vi "ProcCore.vi"(7 "ProcessParams":T1={"DisplayIncrement"=0, "DisplayIncrementRef"=refnum, "Rep .Rate (Hz)"=10.0, "Save"=FALSE, "SW_Average"=0, "Filter"=enum."None", "FilterParams"=variant, "DAQParams"={"TrigDelay"=0.0, "Offset"=0, "Resolution"=-32768, "Range (mV)"=0, "Sample Rate"=100000000.0, "Depth"=16384.0, "Segments"=1}, "Graph"=[], "CmdParams."=variant, "Average(SW)Ref"=refnum, "Calibr.Params"=refnum, "SignalSegmentRef"=refnum, "WriterQueue"=refnum} {"DAQParams"."Segments" min=1 max=1024 step=1; "DAQParams"."Sample Rate" format="%.0p"}, 8 "error in":errorcluster, 9 "SignalBuffer in":refnum<queue>, 10 "CtrlQueue in":refnum<queue>) -> (0 "error out":errorcluster)   [LabVIEW 2013]
uses:
  <instrlib>/AnalogDiscSDKLv/VIs/DWF_Signal.ctl
  ProcessParams.ctl
  ControlDef/ProcessingMode.ctl
  DAQParams.ctl
  DisplayGraph.ctl
  Binning/BinType.ctl
  ControlDef/Average#.ctl
  Files/Signal_Segment.ctl
  ControlDef/Signal.ctl
  ProcessStates.ctl
  <vilib>/Utility/error.llb/DialogType.ctl
  Binning/SpectrumBinning.vi
  MassResolutionCalc/FindMassResolution_Single.vi
  <instrlib>/AnalogDiscSDKLv/AnalogDiscSDKLv.lvlib
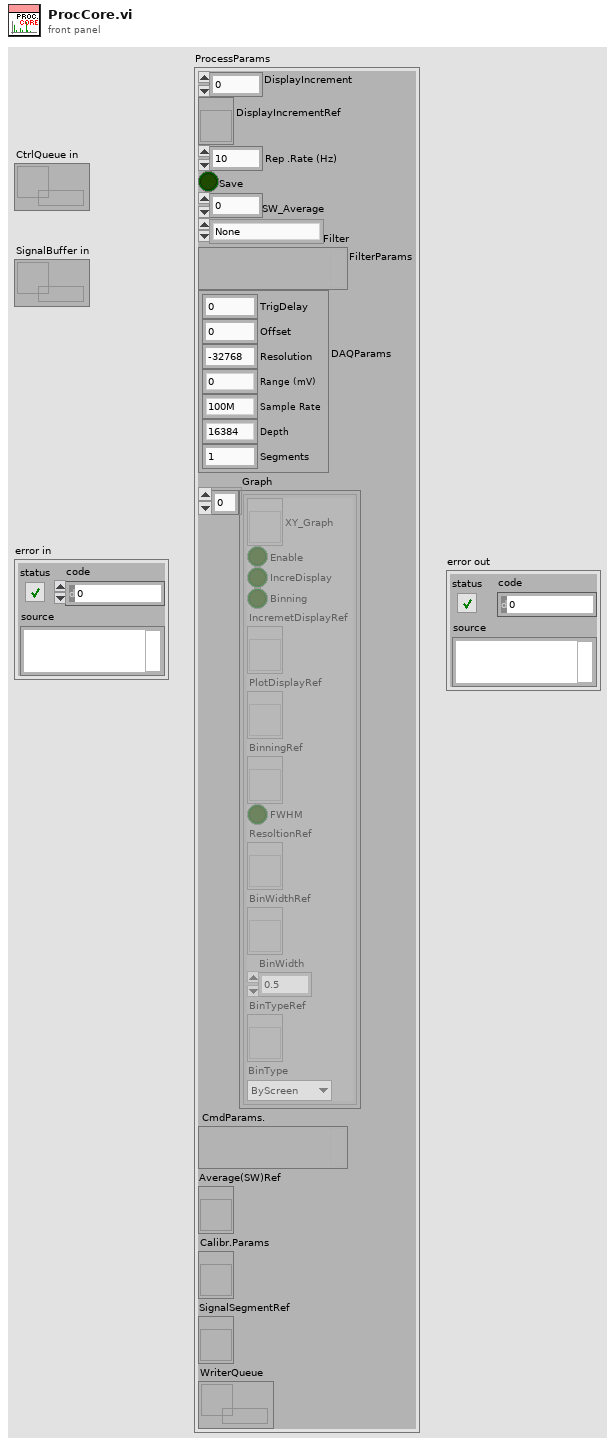
[diagram p1: front panel]
types:
  T1 = typedef "ProcessParams.ctl" = cluster{"DisplayIncrement":u32, "DisplayIncrementRef":refnum<vi>, "Rep .Rate (Hz)":dbl, "Save":bool, "SW_Average":u32, "Filter":T2, "FilterParams":variant, "DAQParams":T3, "Graph":T4[], "CmdParams.":variant, "Average(SW)Ref":refnum<vi>, "Calibr.Params":refnum<vi>, "SignalSegmentRef":refnum<vi>, "WriterQueue":refnum<queue>}
  T2 = typedef "ProcessingMode.ctl" = enum16{"None", "Drop by Threshold", "TDC Simulate", "SetFilter"}
  T3 = typedef "DAQParams.ctl" = cluster{"TrigDelay":dbl, "Offset":i32, "Resolution":i32, "Range (mV)":u32, "Sample Rate":dbl, "Depth":dbl, "Segments":u32}
  T4 = typedef "DisplayGraph.ctl" = cluster{"XY_Graph":refnum<vi>, "Enable":bool, "IncreDisplay":bool, "Binning":bool, "IncremetDisplayRef":refnum<vi>, "PlotDisplayRef":refnum<vi>, "BinningRef":refnum<vi>, "FWHM":bool, "ResoltionRef":refnum<vi>, "BinWidthRef":refnum<vi>, "BinWidth":dbl, "BinTypeRef":refnum<vi>, "BinType":T5}
  T5 = typedef "BinType.ctl" = enum16{"ByTime", "ByScreen", "ByMass", "ToUnitMass"}
  T6 = typedef "ProcessStates.ctl" = enum16{"Initialize", "Normal", "Display", "Write2Buffer", "CalcMzArray", "StartSave", "StopSave", "ConfigChanged", "EndOfLine", "SetFilterParams", "SetGraphsEnable", "SetAcquisitionParams", "ChangeDisplayIncrement", "ChangeRepRate", "SetWriterRef", "Quit", "StartOfLine"}
  T7 = typedef "Signal_Segment.ctl" = cluster{"SampleRate":dbl, "TrigDelay":dbl, "SpecLength":dbl, "DAQ_Range":dbl, "Average#":i32, "Position":dbl[], "Spectrum":sgl[], "Calibr.":dbl[], "Pressure":dbl, "Desp_LaserEnergy":dbl, "PI_LaserEnergy":dbl, "Voltages Table":sgl[][], "ProcMode":T2, "Threshold":dbl, "Comment":string, "TickCount":dbl, "Time Stamp":timestamp}
  T8 = typedef "Average#.ctl" = u16
  T9 = typedef "Signal.ctl" = cluster{"Command":T6, "Params":variant}
  T10 = typedef "AnalogDiscSDKLv.lvlib/DWF_Signal.ctl" = cluster{"tickcount":u32, "Signal":sgl[][], "SecondaryData":dbl[], "Flag":enum16{"Normal", "MultiRecStart", "MultiRecEnd", "Reserved1", "Reserved2", "Reserved3"}}
  T11 = enum16{"Normal", "MultiRecStart", "MultiRecEnd", "Reserved1", "Reserved2", "Reserved3"}
  T12 = typedef "DialogType.ctl" = u16
  T13 = cluster{"WriterQueue":refnum<queue>, "feedback queue":refnum<queue>}
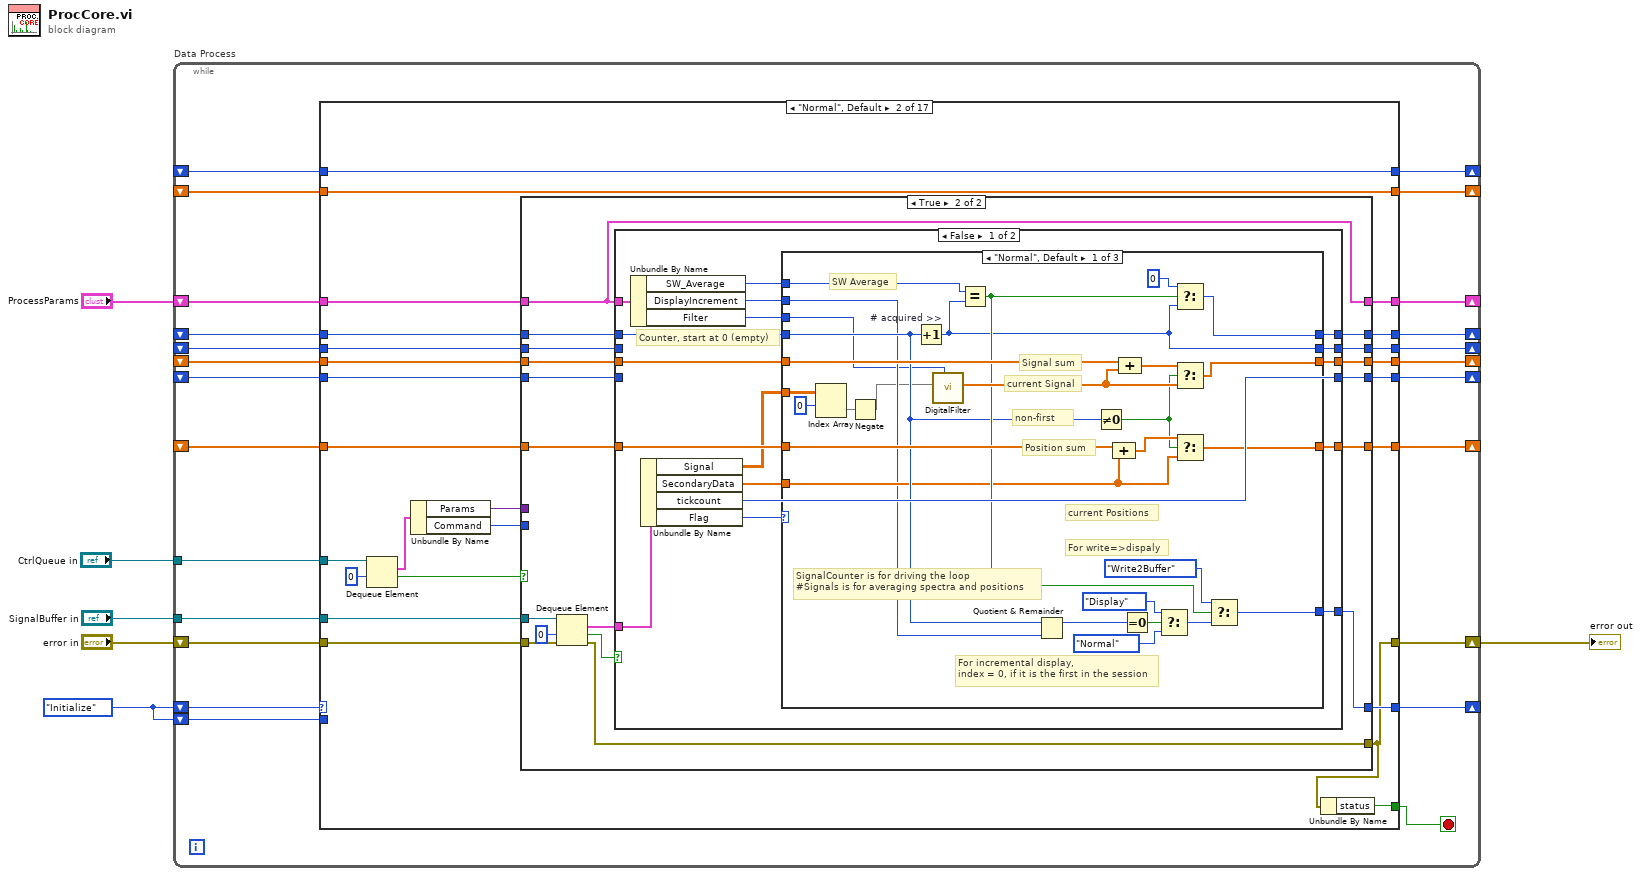
[diagram p0: block diagram]
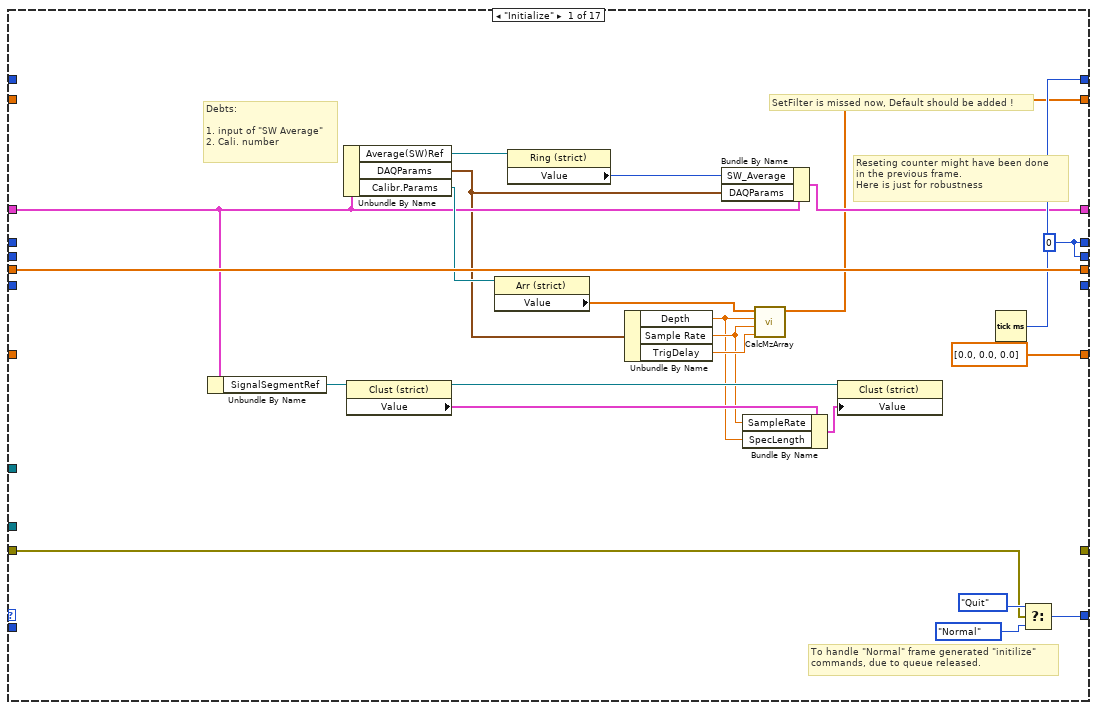
[diagram p2: hidden frame]
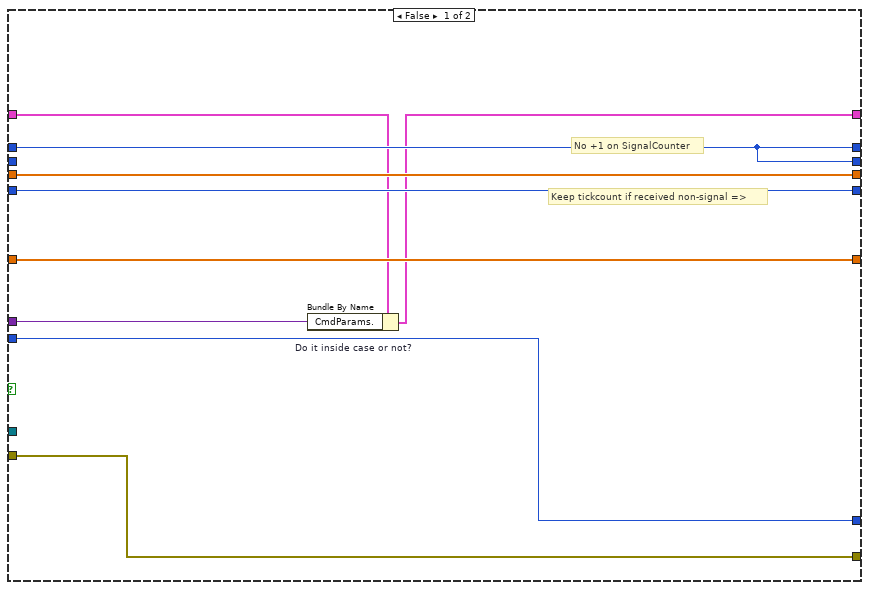
[diagram p3: hidden frame]
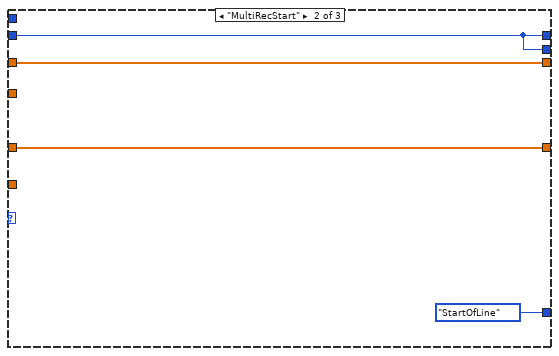
[diagram p4: hidden frame]
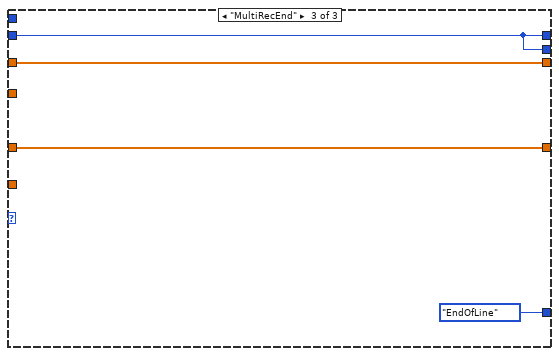
[diagram p5: hidden frame]
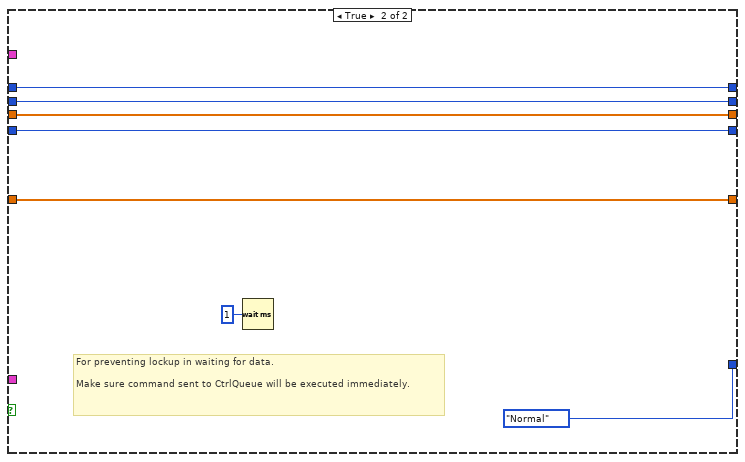
[diagram p6: hidden frame]
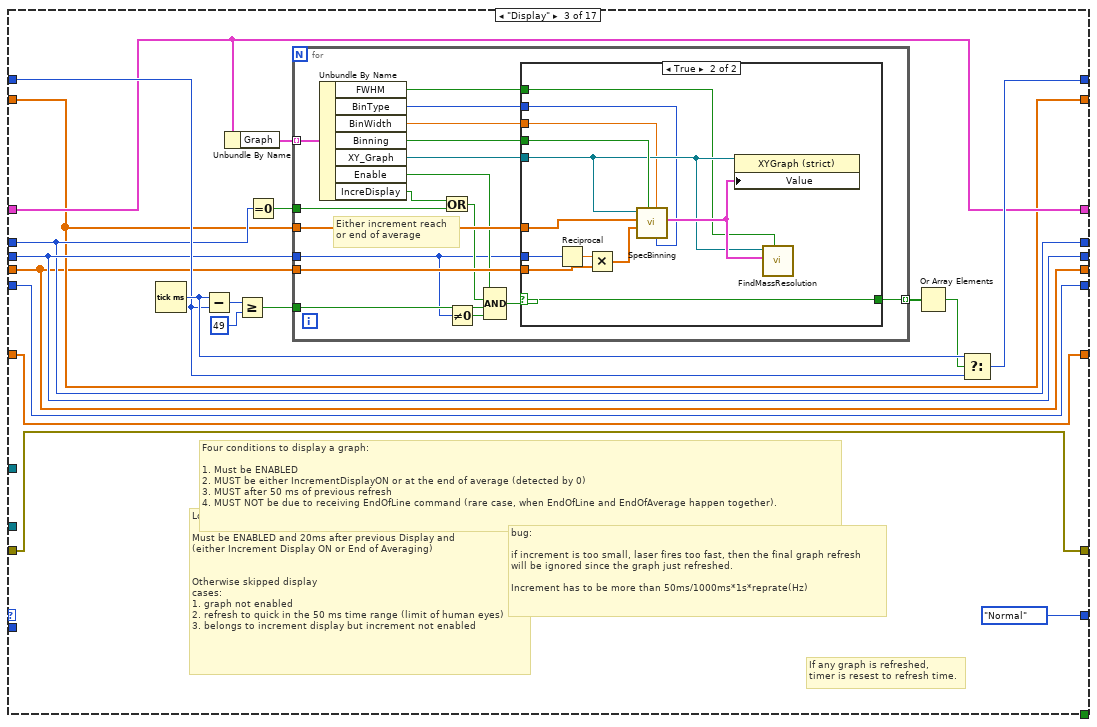
[diagram p7: hidden frame]
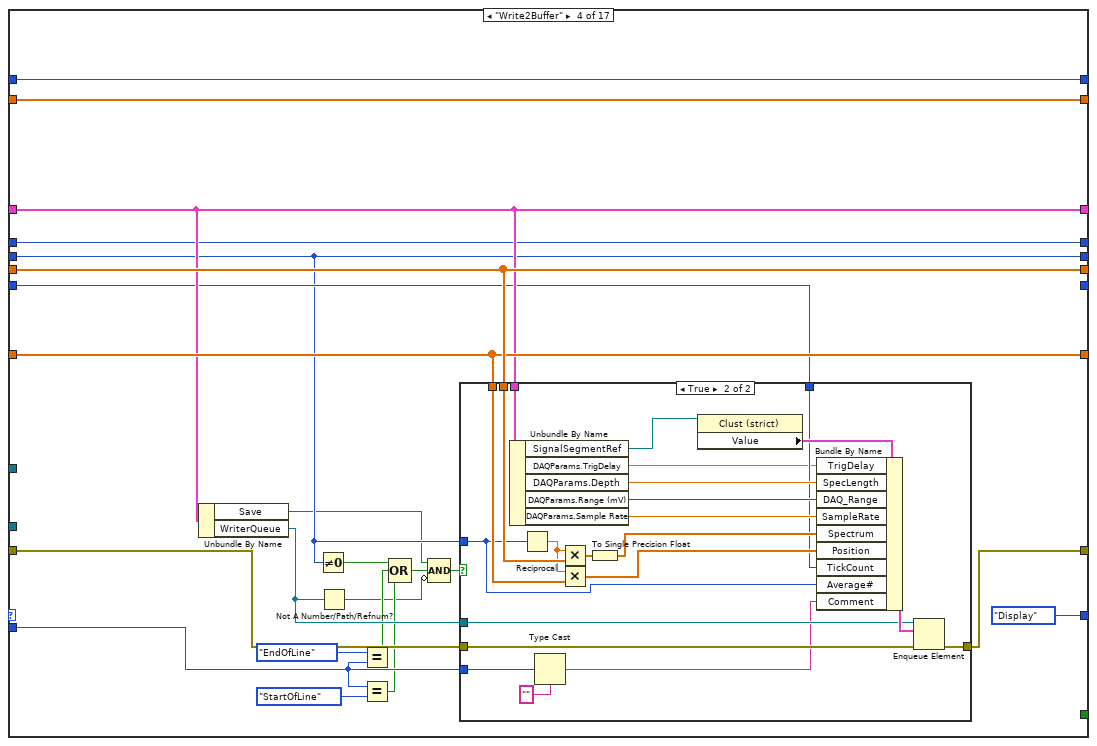
[diagram p9: hidden frame]
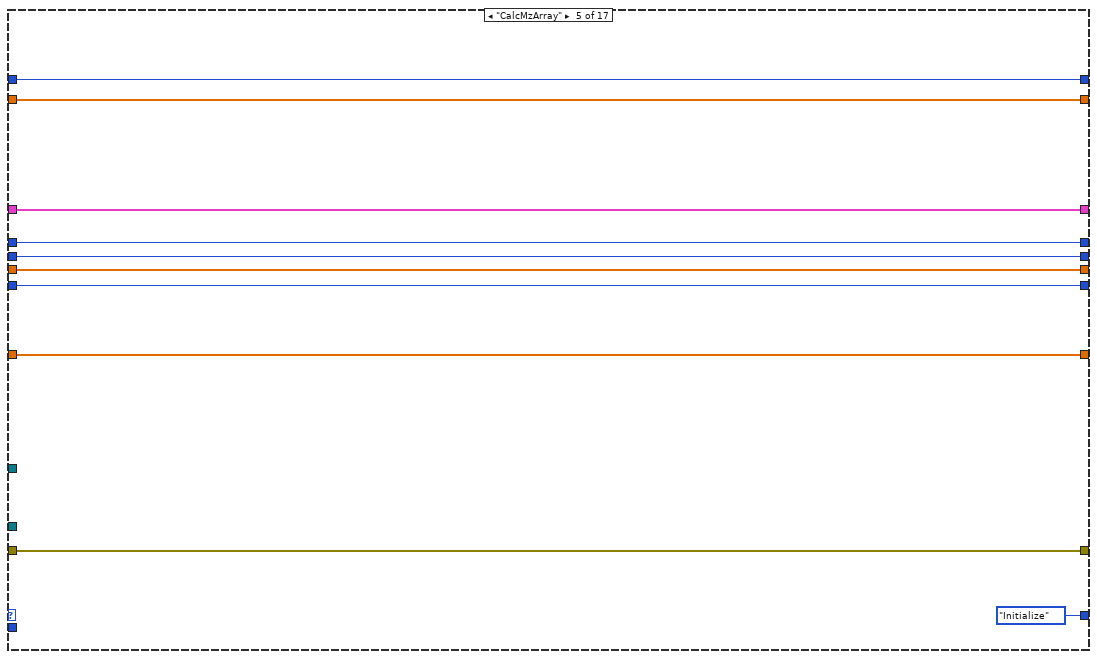
[diagram p11: hidden frame]
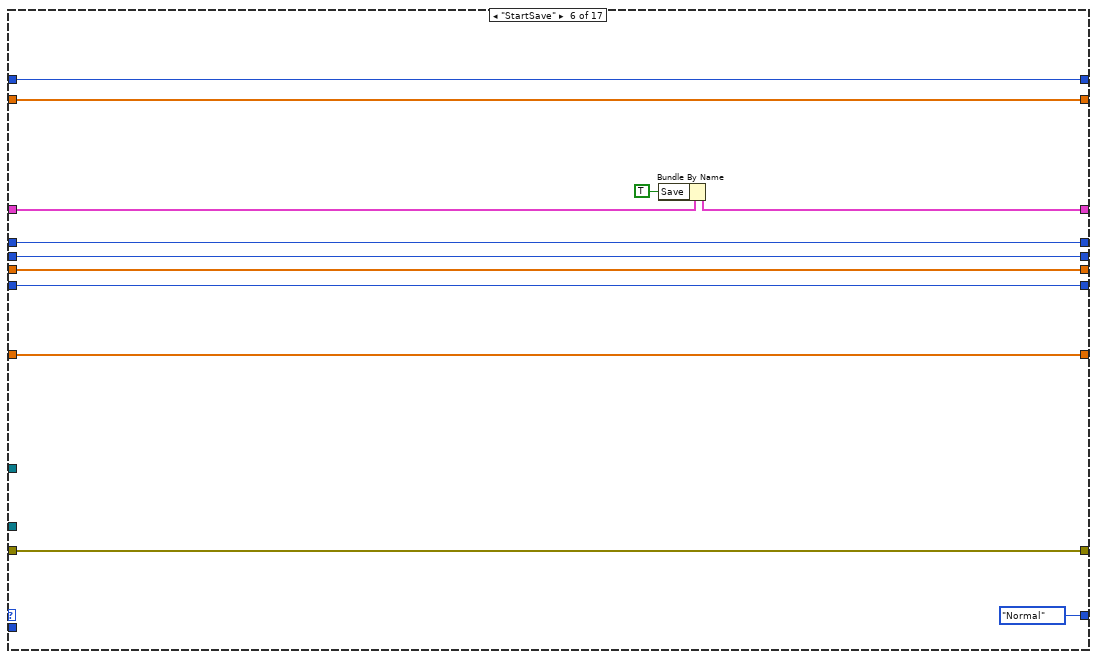
[diagram p12: hidden frame]
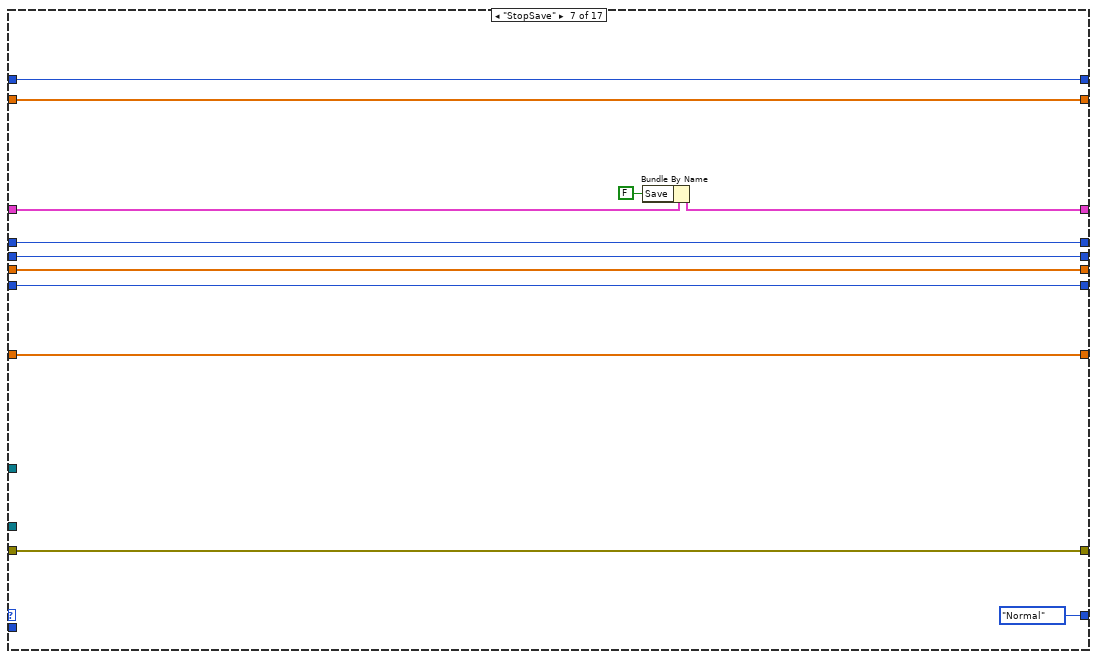
[diagram p13: hidden frame]
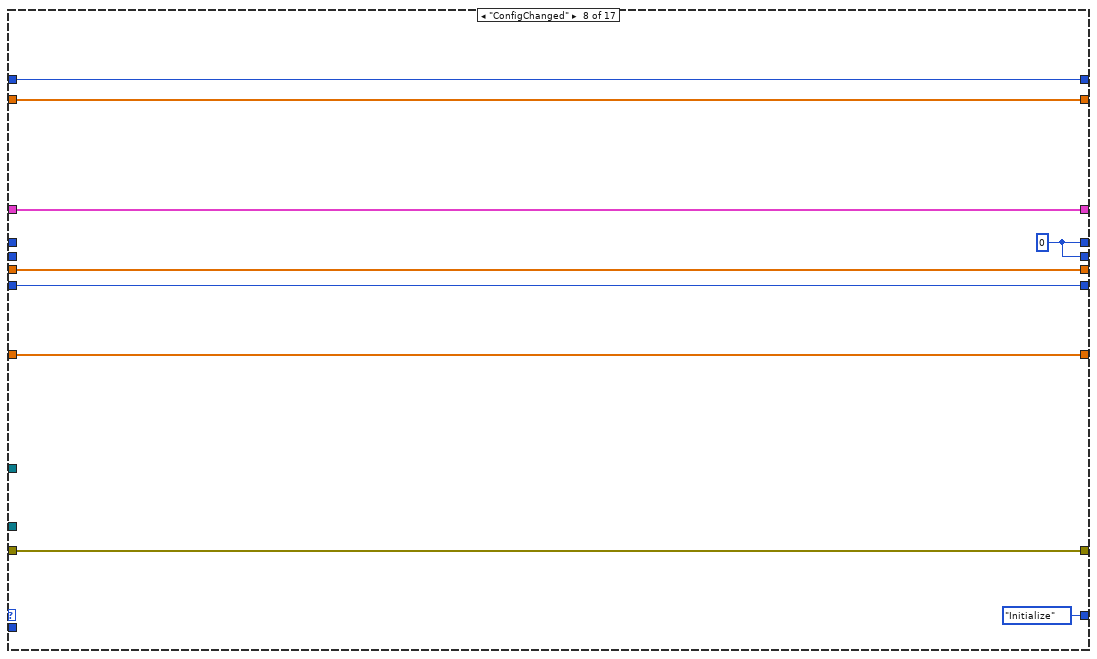
[diagram p14: hidden frame]
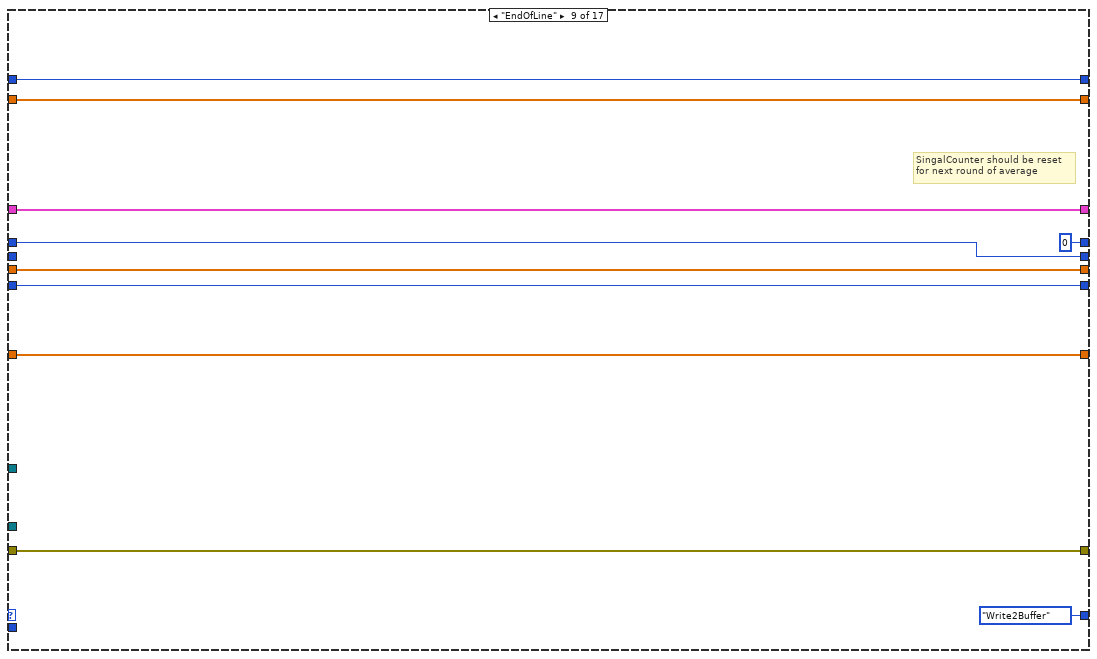
[diagram p15: hidden frame]
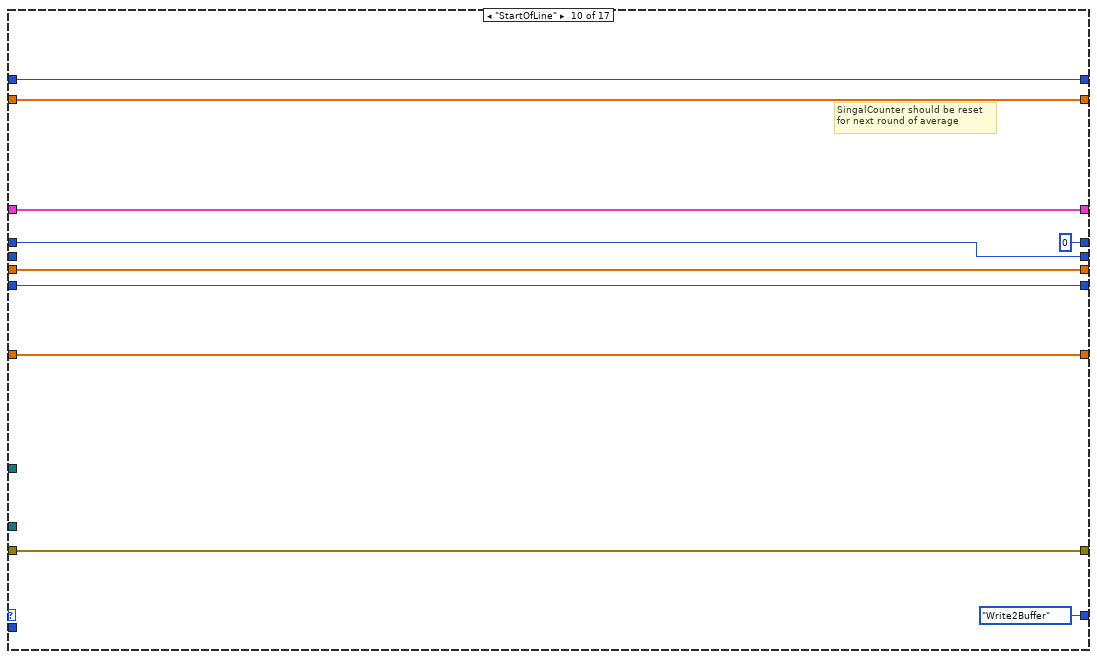
[diagram p16: hidden frame]
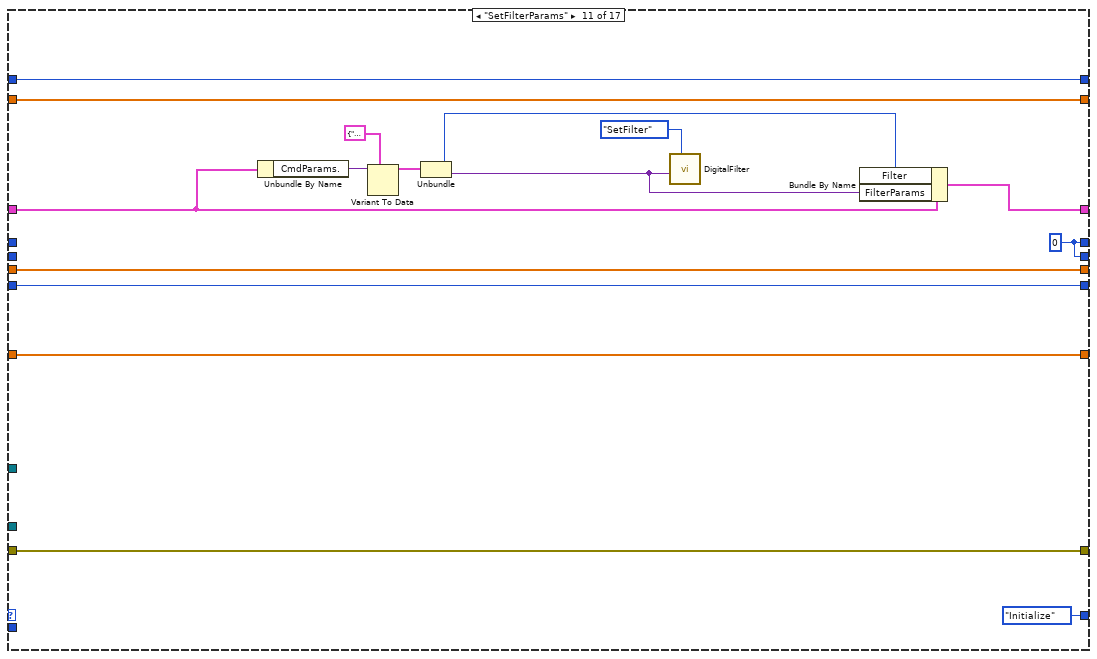
[diagram p17: hidden frame]
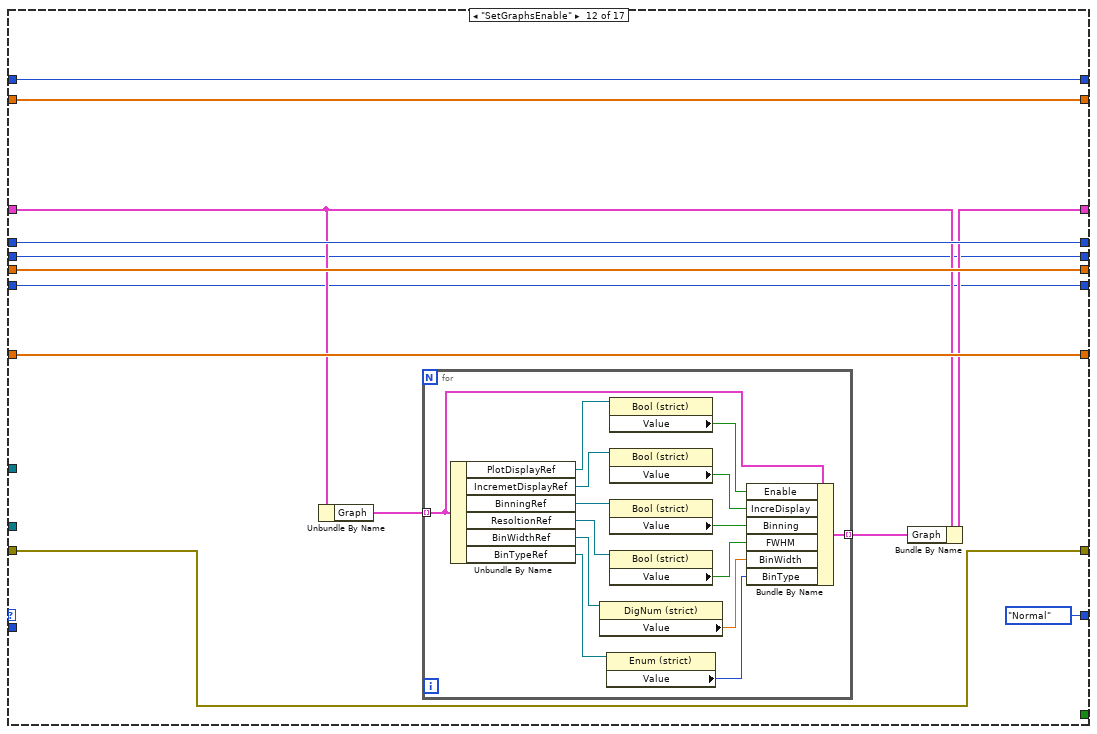
[diagram p18: hidden frame]
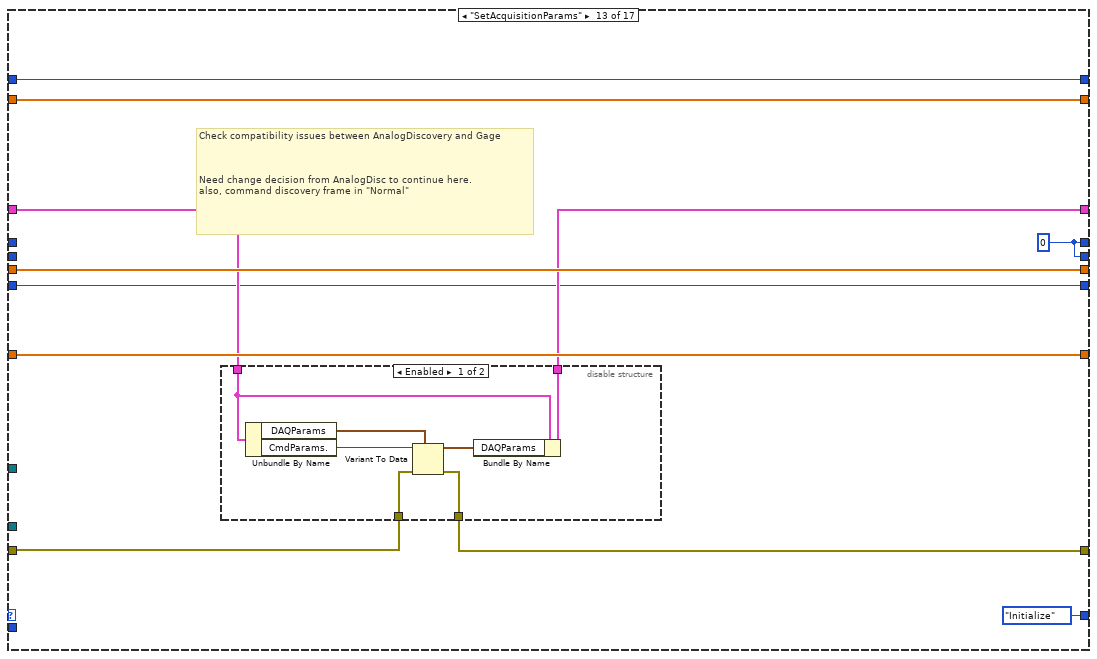
[diagram p19: hidden frame]
diagram:
  w3 = ProcessStates."Initialize"
  n1 = while "Data Process" {
    tunnel: "SignalBuffer in" -> [w30]
    shift-right: [w24] -> _
    shift-left: _ -> [w28]
    shift-right: [w26] -> _
    shift-left: _ -> [w27]
    shift-right: [w25] -> w4
    shift-left: "error in" -> [w29]
    shift-right: [w16] -> _
    shift-left: _ -> [w22]
    shift-right: [w17] -> _
    shift-left: _ -> [w21]
    shift-right: [w14] -> _
    shift-left: _ -> [w15]
    shift-right: [w19] -> _
    shift-left: "ProcessParams" -> [w20]
    shift-right: [w18] -> _
    shift-left: w3 -> [w13]
    shift-left: w3 -> [w12]
    shift-right: [w11] -> _
    shift-left: _ -> [w10]
    shift-right: [w9] -> _
    shift-left: _ -> [w8]
    tunnel: "CtrlQueue in" -> [w7]
    stop <- w23 stop-if-true
    n2 = case shown="\"Normal\", Default" w13 {
      tunnel: w30 -> [_ w60 _ _ _ _ _ _ _ _ _ _ _ _ _ _ _]
      tunnel: w29 -> [w41 w58 w184 w233 w267 w279 w291 w300 w310 w320 w336 w349 w369 w401 w427 w452 w474]
      tunnel: w28 -> [w53 w74 w166 w231 w266 w278 w290 w299 w309 w319 w335 w348 w374 w400 w426 w457 w481]
      tunnel: w27 -> [_ w78 w180 w230 w268 w280 w292 w301 w311 w321 w337 w350 w375 w402 w428 w458 w482]
      tunnel: [dbl[] [0.0, 0.0, 0.0] w72 w180 w230 w268 w280 w292 w301 w311 w321 w337 w350 w375 w402 w428 w458 w482] -> w26
      tunnel: [_ w59 w184 w232 w267 w279 w291 w300 w310 w320 w336 w349 w368 w401 w427 w442 w474] -> w25
      tunnel: [w53 w75 w166 w231 w266 w278 w290 w299 w309 w319 w335 w348 w374 w400 w426 w457 w481] -> w24
      tunnel: [_ w69 _ _ _ _ _ _ _ _ _ _ _ _ _ _ TRUE] -> w23
      tunnel: w22 -> [_ w77 w176 w235 w264 w275 w287 w297 w307 w317 w334 w346 w373 w398 w424 w456 w478]
      tunnel: w21 -> [_ w70 w170 w227 w265 w276 w288 _ w304 w314 _ w347 _ w399 w425 _ w479]
      tunnel: w15 -> [_ w76 w167 w234 w261 w274 w286 w296 w306 w316 w333 w345 w372 w397 w423 w455 w477]
      tunnel: w20 -> [w40 w56 w169 w228 w262 w277 w289 w298 w308 w318 w329 w342 w367 w394 w420 w451 w480]
      tunnel: [w49 w55 w169 w228 w262 w273 w285 w298 w308 w318 w332 w344 w370 w393 w415 w453 w480] -> w19
      tunnel: [w42 w73 ProcessStates."Normal" ProcessStates."Display" ProcessStates."Initialize" ProcessStates."Normal" ProcessStates."Normal" ProcessStates."Initialize" ProcessStates."Write2Buffer" ProcessStates."Write2Buffer" ProcessStates."Initialize" ProcessStates."Normal" ProcessStates."Initialize" ProcessStates."Normal" ProcessStates."Normal" ProcessStates."Normal" ProcessStates."Quit"] -> w18
      tunnel: [w33 w71 w170 w227 w265 w276 w288 w294 u32 0 ("t") u32 0 ("t") w323 w347 w366 w399 w425 w450 w479] -> w17
      tunnel: [w51 w77 w177 w235 w264 w275 w287 w297 w307 w317 w334 w346 w373 w398 w424 w456 w478] -> w16
      tunnel: [w32 w76 w167 w234 w261 w274 w286 w296 w306 w316 w333 w345 w372 w397 w423 w455 w477] -> w14
      tunnel: w12 -> [_ _ _ w219 _ _ _ _ _ _ _ _ _ _ _ _ _]
      tunnel: [w33 w68 w172 w225 w260 w270 w282 w294 w304 w314 w323 w339 w366 w396 w422 w450 w473] -> w11
      tunnel: w10 -> [_ w54 w172 w225 w260 w270 w282 _ _ _ _ w339 _ w396 w422 _ w473]
      tunnel: [_ w67 w168 _ w259 w269 w281 w293 w302 w312 w322 w338 w365 w392 w418 w449 _] -> w9
      tunnel: w8 -> [_ w66 w168 w226 w259 w269 w281 w293 w302 w312 w322 w338 w365 w392 w418 w449 _]
      tunnel: w7 -> [_ w64 _ _ _ _ _ _ _ _ _ _ _ _ _ _ _]
      frame "Initialize" {
        w33 = u32 0 ("t")
        # "SetFilter is missed now, Default should be added !"
        # "Reseting counter might have been done\nin the previous frame.\nHere is just for robustness"
        # "To handle \"Normal\" frame generated \"initilize\"\ncommands, due to queue released."
        # "Debts:\n\n1. input of \"SW Average\"\n2. Cali. number"
        n3 = Unbundle By Name(w40) -> ("SignalSegmentRef"=w39:refnum<vi>)
        n4 = Unbundle By Name(w40) -> ("Average(SW)Ref"=w48:refnum<vi>, "DAQParams"=w31:T3, "Calibr.Params"=w45:refnum<vi>)
        n5 = property class="Clust (strict)"(reference=w39) -> (reference out=w38:refnum<vi>, "Value"=w37:T7)  [unwired: 1 in, 1 out]
        n6 = property class="Arr (strict)"(reference=w45) -> ("Value"=w46:dbl[])  [unwired: 1 in, 2 out]
        n7 = property class="Ring (strict)"(reference=w48) -> ("Value"=w47:T8)  [unwired: 1 in, 2 out]
        n8 = Unbundle By Name(w31) -> ("Depth"=w34:dbl, "Sample Rate"=w35:dbl, "TrigDelay"=w50:dbl)
        n9 = Bundle By Name(cluster=w40, "SW_Average"=w47, "DAQParams"=w31) -> (w49:T1)
        n10 = Bundle By Name(cluster=w37, "SampleRate"=w35, "SpecLength"=w34) -> (w36:T7)
        n11 = call "CalcMzArray.vi"("TrigDelay"=w50, "Sample Rate"=w35, "Depth"=w34, "mzCali. (a/b/c)"=w46) -> ("mzArray"=w32:dbl[])  [unwired: 7 in]
        n12 = property class="Clust (strict)"(reference=w38, "Value"=w36) -> ()  [unwired: 1 in, 2 out]
        n13 = Tick Count (ms)() -> (millisecond timer value=w51:u32)
        n14 = Select(t=ProcessStates."Quit", s=w41, f=ProcessStates."Normal") -> (s? t:f=w42:T6)
      }
      frame "Normal", Default {
        # "Normal condition, waiting data coming, choose next frame"
        n15 = Dequeue Element(queue=w64, timeout in ms (-1)=0) -> (element=w63:T9, timed out?=w61:bool)  [unwired: 1 in, 2 out]
        n16 = Unbundle By Name(w63) -> ("Params"=w57:variant, "Command"=w62:T6)
        n17 = case shown="True" w61 {
          tunnel: w78 -> [w87 w105]
          tunnel: [w86 w104] -> w75
          tunnel: w74 -> [w86 w103]
          tunnel: [w85 w100] -> w73
          tunnel: w62 -> [w85 _]
          tunnel: [w87 w102] -> w72
          tunnel: [w84 w101] -> w71
          tunnel: w70 -> [w84 w98]
          tunnel: [w84 w99] -> w68
          tunnel: [w83 w97] -> w67
          tunnel: w66 -> [w83 w89]
          tunnel: w56 -> [w80 w88]
          tunnel: w60 -> [_ w96]
          tunnel: [w82 w94] -> w59
          tunnel: w58 -> [w82 w93]
          tunnel: w57 -> [w81 _]
          tunnel: [w79 w88] -> w55
          tunnel: w54 -> [_ w90]
          frame False {
            # "Keep tickcount if received non-signal =>"
            # "No +1 on SignalCounter"
            # "Received command other than signal"
            n18 = Bundle By Name "Do it inside case or not?"(cluster=w80, "CmdParams."=w81) -> (w79:T1)
          }
          frame True {
            # "Normal condition: summing"
            n19 = Dequeue Element(queue=w96, timeout in ms (-1)=0, error in (no error)=w93) -> (element=w95:T10, timed out?=w91:bool, error out=w94:errorcluster)  [unwired: 1 out]
            n20 = case shown="False" w91 {
              tunnel: w105 -> [w122 w161]
              tunnel: [w121 w163] -> w104
              tunnel: w103 -> [w120 w163]
              tunnel: [w119 w161] -> w102
              tunnel: [w118 w162] -> w101
              tunnel: [w117 ProcessStates."Normal"] -> w100
              tunnel: [w116 w160] -> w99
              tunnel: w98 -> [w115 w162]
              tunnel: [w114 w159] -> w97
              tunnel: w95 -> [w108 _]
              tunnel: w88 -> [w107 _]
              tunnel: w90 -> [_ w160]
              tunnel: w89 -> [_ w159]
              frame False {
                # "Counter, start at 0 (empty)"
                n21 = Unbundle By Name(w107) -> ("SW_Average"=w109:u32, "DisplayIncrement"=w111:u32, "Filter"=w110:T2)
                n22 = Unbundle By Name(w108) -> ("Signal"=w112:sgl[][], "SecondaryData"=w113:dbl[], "tickcount"=w114:u32, "Flag"=w106:T11)
                n23 = case shown="\"Normal\", Default" w106 {
                  tunnel: w122 -> [w150 w151 w157]
                  tunnel: [w123 w152 w156] -> w121
                  tunnel: w120 -> [w148 w152 w156]
                  tunnel: [w124 w151 w157] -> w119
                  tunnel: [w142 w153 w155] -> w118
                  tunnel: [w139 ProcessStates."StartOfLine" ProcessStates."EndOfLine"] -> w117
                  tunnel: [w134 w153 w155] -> w116
                  tunnel: w115 -> [w133 w153 w155]
                  tunnel: w113 -> [w130 _ _]
                  tunnel: w112 -> [w129 _ _]
                  tunnel: w111 -> [w128 _ _]
                  tunnel: w110 -> [w127 _ _]
                  tunnel: w109 -> [w126 _ _]
                  frame "Normal", Default {
                    # "SignalCounter is for driving the loop\n#Signals is for averaging spectra and positions"
                    # "SW Average"
                    # "For write=>dispaly"
                    # "For incremental display,\nindex = 0, if it is the first in the session"
                    # "non-first"
                    # "Signal sum"
                    # "current Signal"
                    # "Position sum"
                    # "current Positions"
                    n24 = Index Array(array=w129, index (row)=0) -> (element=w132:sgl[])  [unwired: 1 in]
                    n25 = Negate(x=w132) -> (-x=w125:sgl[])
                    n26 = Increment "# acquired >>"(x=w133) -> (x+1=w134:u32)
                    n27 = call "DigitalFilter.vi"("Filter"=w127, "Original Data"=w125) -> ("Output"=w141:dbl[])  [unwired: 9 in]
                    n28 = Equal?(x=w126, y=w134) -> (x = y?=w140:bool)
                    n29 = Quotient & Remainder(x=w133, y=w128) -> (x-y*floor(x/y)=w144:u32)  [unwired: 1 out]
                    n30 = Not Equal To 0?(x=w133) -> (x != 0?=w137:bool)
                    n31 = Compound Arithmetic op=ADD(w150, w130) -> (w143:dbl[])
                    n32 = Compound Arithmetic op=ADD(w148, w141) -> (w149:dbl[])
                    n33 = Equal To 0?(x=w144) -> (x = 0?=w145:bool)
                    n34 = Select(t=ProcessStates."Display", s=w145, f=ProcessStates."Normal") -> (s? t:f=w135:T6)
                    n35 = Select(t=u32 0, s=w140, f=w134) -> (s? t:f=w142:u32)
                    n36 = Select(t=w149, s=w137, f=w141) -> (s? t:f=w123:dbl[])
                    n37 = Select(t=w143, s=w137, f=w130) -> (s? t:f=w124:dbl[])
                    n38 = Select(t=ProcessStates."Write2Buffer" ("f"), s=w140, f=w135) -> (s? t:f=w139:T6)
                  }
                  frame "MultiRecStart" {
                  }
                  frame "MultiRecEnd" {
                  }
                }
              }
              frame True {
                # "For preventing lockup in waiting for data. \n\nMake sure command sent to CtrlQueue will be executed immediately."
                n39 = Wait (ms)(milliseconds to wait=u32 1) -> ()  [unwired: 1 out]
              }
            }
          }
        }
        n40 = Unbundle By Name(w59) -> ("status"=w69:bool)
      }
      frame "Display" {
        # "bug:\n\nif increment is too small, laser fires too fast, then the final graph refresh\nwill be ignored since the graph just refreshed.\n\nIncrement has to be more than 50ms/1000ms*1s*reprate(Hz)"
        # "Four conditions to display a graph:\n\n1. Must be ENABLED\n2. MUST be either IncrementDisplayON or at the end of average (detected by 0)\n3. MUST after 50 ms of previous refresh\n4. MUST NOT be due to receiving EndOfLine command (rare case, when EndOfLine and EndOfAverage happen together)."
        # "If any graph is refreshed, \ntimer is resest to refresh time."
        # "Logic to Diskplay:\n\nMust be ENABLED and 20ms after previous Display and \n(either Increment Display ON or End of Averaging)\n\n\nOtherwise skipped display\ncases:\n1. graph not enabled\n2. refresh to quick in the 50 ms time range (limit of human eyes)\n3. belongs to increment display but increment not enabled"
        n41 = Tick Count (ms)() -> (millisecond timer value=w178:u32)
        n42 = Subtract(x=w178, y=w176) -> (x-y=w182:u32)
        n43 = Unbundle By Name(w169) -> ("Graph"=w183:T4[])
        n44 = Greater Or Equal?(x=w182, y=u32 49) -> (x >= y?=w179:bool)
        n45 = Equal To 0?(x=w170) -> (x = 0?=w171:bool)
        n46 = for {
          tunnel: w183 -> [w201] mode=indexing
          tunnel: w167 -> [w199]
          tunnel: w166 -> [w198]
          tunnel: w179 -> [w195]
          tunnel: [w192] -> w174 mode=indexing
          tunnel: w172 -> [w188]
          tunnel: w171 -> [w191]
          # "Either increment reach \nor end of average"
          n47 = Unbundle By Name(w201) -> ("FWHM"=w187:bool, "BinType"=w185:T5, "BinWidth"=w186:dbl, "Binning"=w190:bool, "XY_Graph"=w200:refnum<vi>, "Enable"=w196:bool, "IncreDisplay"=w193:bool)
          n48 = Or(x=w193, y=w191) -> (x .or. y?=w194:bool)
          n49 = Not Equal To 0?(x=w188) -> (x != 0?=w189:bool)
          n50 = Compound Arithmetic op=AND(w196, w194, w195, w189) -> (w197:bool)
          n51 = case shown="True" w197 {
            selector: w197 -> [_ w208]
            tunnel: w200 -> [_ w205]
            tunnel: w199 -> [_ w213]
            tunnel: w198 -> [_ w211]
            tunnel: w188 -> [_ w209]
            tunnel: [_ w208] -> w192
            tunnel: w190 -> [_ w207]
            tunnel: w187 -> [_ w204]
            tunnel: w186 -> [_ w203]
            tunnel: w185 -> [_ w202]
            frame False {
            }
            frame True {
              n52 = Reciprocal(x=w209) -> (1/x=w212:dbl)
              n53 = Multiply(x=w212, y=w211) -> (x*y=w210:dbl[])
              n54 = call-poly "SpecBinning.vi"("BinType"=w202, "BinWidth"=w203, "Binning (T)"=w207, "Signal"=w210, "m/z Array"=w213, "GraphRef."=w205) -> ("BinnedSpectrum"=w206:cluster{"m/z Array":dbl[], "Signal":dbl[]})  [unwired: 4 in, 1 out]
              n55 = property class="XYGraph (strict)"(reference=w205, "Value"=w206) -> ()  [unwired: 1 in, 2 out]
              n56 = call-poly "FindMassResolution.vi"("EnableResDisplay"=w204, "BinnedSpectrum"=w206, "GraphRef"=w205) -> ()  [unwired: 7 in, 2 out]
            }
          }
        }
        n57 = Or Array Elements(Boolean array=w174) -> (logical OR=w173:bool)
        n58 = Select(t=w178, s=w173, f=w176) -> (s? t:f=w177:u32)
      }
      frame "Write2Buffer" {
        # "Send averaged spectra to buffer(writer), and continue to graph display"
        n59 = Unbundle By Name(w228) -> ("Save"=w215:bool, "WriterQueue"=w224:refnum<queue>)
        n60 = Not Equal To 0?(x=w225) -> (x != 0?=w214:bool)
        n61 = Not A Number/Path/Refnum?(number/path/refnum=w224) -> (NaN/Path/Refnum?=w216:bool)
        n62 = Equal?(x=ProcessStates."EndOfLine", y=w219) -> (x = y?=w221:bool)
        n63 = Equal?(x=w219, y=ProcessStates."StartOfLine" ("x")) -> (x = y?=w218:bool)
        n64 = Compound Arithmetic op=OR(w214, w221, w218) -> (w223:bool)
        n65 = Compound Arithmetic op=AND(w215, w223, invert w216) -> (w217:bool)
        n66 = case shown="True" w217 {
          tunnel: w224 -> [_ w257]
          tunnel: w233 -> [w236 w256]
          tunnel: [w236 w255] -> w232
          tunnel: w231 -> [_ w254]
          tunnel: w230 -> [_ w250]
          tunnel: w225 -> [_ w238]
          tunnel: w228 -> [_ w248]
          tunnel: w219 -> [_ w237]
          tunnel: w226 -> [_ w240]
          frame False {
          }
          frame True {
            n67 = Unbundle By Name(w248) -> ("SignalSegmentRef"=w244:refnum<vi>, "DAQParams.TrigDelay"=w239:dbl, "DAQParams.Depth"=w245:dbl, "DAQParams.Range (mV)"=w246:u32, "DAQParams.Sample Rate"=w247:dbl)
            n68 = Reciprocal(x=w238) -> (1/x=w251:dbl)
            n69 = Type Cast(type="", x=w237) -> (*(type *) &x=w242:string)
            n70 = Multiply(x=w251, y=w254) -> (x*y=w253:dbl[])
            n71 = Multiply(x=w251, y=w250) -> (x*y=w252:dbl[])
            n72 = To Single Precision Float(number=w253) -> (single precision float=w249:sgl[])
            n73 = property class="Clust (strict)"(reference=w244) -> ("Value"=w243:T7)  [unwired: 1 in, 2 out]
            n74 = Bundle By Name(cluster=w243, "TrigDelay"=w239, "SpecLength"=w245, "DAQ_Range"=w246, "SampleRate"=w247, "Spectrum"=w249, "Position"=w252, "TickCount"=w240, "Average#"=w238, "Comment"=w242) -> (w258:T7)
            n75 = Enqueue Element(queue=w257, element=w258, error in (no error)=w256) -> (error out=w255:errorcluster)  [unwired: 1 in, 2 out]
          }
        }
      }
      frame "CalcMzArray" {
      }
      frame "StartSave" {
        n76 = Bundle By Name(cluster=w277, "Save"=TRUE) -> (w273:T1)
      }
      frame "StopSave" {
        n77 = Bundle By Name(cluster=w289, "Save"=FALSE) -> (w285:T1)
      }
      frame "ConfigChanged" {
        w294 = u32 0
      }
      frame "EndOfLine" {
        # "SingalCounter should be reset\nfor next round of average"
        # "FlushBuffer, reset averager"
      }
      frame "StartOfLine" {
        # "SingalCounter should be reset\nfor next round of average"
        # "FlushBuffer, reset averager"
      }
      frame "SetFilterParams" {
        w323 = u32 0
        n78 = Unbundle By Name(w329) -> ("CmdParams."=w328:variant)
        n79 = Variant To Data(type=cluster{"Processing Mode":T2, "Variant":variant} {"Processing Mode"=enum."None", "Variant"=variant} ("cluster"), Variant=w328) -> (data=w326:cluster{"Processing Mode":T2, "Variant":variant})  [unwired: 1 in, 1 out]
        n80 = Unbundle(w326) -> ("Processing Mode"=w325:T2, "Variant"=w324:variant)
        n81 = call "DigitalFilter.vi"("Filter"=ProcessingMode."SetFilter", "FilterParams"=w324) -> ()  [unwired: 9 in, 1 out]
        n82 = Bundle By Name(cluster=w329, "Filter"=w325, "FilterParams"=w324) -> (w332:T1)
      }
      frame "SetGraphsEnable" {
        n83 = Unbundle By Name(w342) -> ("Graph"=w341:T4[])
        n84 = for {
          tunnel: w341 -> [w364] mode=indexing
          tunnel: [w357] -> w340 mode=indexing
          n85 = Unbundle By Name(w364) -> ("PlotDisplayRef"=w363:refnum<vi>, "IncremetDisplayRef"=w362:refnum<vi>, "BinningRef"=w361:refnum<vi>, "ResoltionRef"=w355:refnum<vi>, "BinWidthRef"=w353:refnum<vi>, "BinTypeRef"=w352:refnum<vi>)
          n86 = property class="DigNum (strict)"(reference=w353) -> ("Value"=w354:dbl)  [unwired: 1 in, 2 out]
          n87 = property class="Enum (strict)"(reference=w352) -> ("Value"=w351:T5)  [unwired: 1 in, 2 out]
          n88 = property class="Bool (strict)"(reference=w363) -> ("Value"=w360:bool)  [unwired: 1 in, 2 out]
          n89 = property class="Bool (strict)"(reference=w362) -> ("Value"=w359:bool)  [unwired: 1 in, 2 out]
          n90 = property class="Bool (strict)"(reference=w361) -> ("Value"=w358:bool)  [unwired: 1 in, 2 out]
          n91 = property class="Bool (strict)"(reference=w355) -> ("Value"=w356:bool)  [unwired: 1 in, 2 out]
          n92 = Bundle By Name(cluster=w364, "Enable"=w360, "IncreDisplay"=w359, "Binning"=w358, "FWHM"=w356, "BinWidth"=w354, "BinType"=w351) -> (w357:T4)
        }
        n93 = Bundle By Name(cluster=w342, "Graph"=w340) -> (w344:T1)
      }
      frame "SetAcquisitionParams" {
        w366 = u32 0 ("t")
        # "Check compatibility issues between AnalogDiscovery and Gage\n\n\n\nNeed change decision from AnalogDisc to continue here. \nalso, command discovery frame in \"Normal\""
        n94 = disable-structure shown="Enabled" {
          disable-tunnel: [w382 w383] -> w370
          disable-tunnel: w369 -> [w380 _]
          disable-tunnel: [w379 _] -> w368
          disable-tunnel: w367 -> [w378 w383]
          frame Enabled {
            n95 = Unbundle By Name(w378) -> ("DAQParams"=w376:T3, "CmdParams."=w377:variant)
            n96 = Variant To Data(error in=w380, type=w376, Variant=w377) -> (data=w381:T3, error out=w379:errorcluster)
            n97 = Bundle By Name(cluster=w378, "DAQParams"=w381) -> (w382:T1)
          }
          frame Disabled {
          }
        }
      }
      frame "ChangeDisplayIncrement" {
        # "DisplayIncrement has to have a fail-safe value, such as 50"
        # "Should add increment range check \n\nincrement has to be larger than 50/1000*reprate(Hz)"
        n98 = Unbundle By Name(w394) -> ("Rep .Rate (Hz)"=w391:dbl, "DisplayIncrementRef"=w386:refnum<vi>, "DisplayIncrement"=w384:u32)
        n99 = property class="DigNum (strict)"(reference=w386) -> (reference out=w387:refnum<vi>, "Value"=w385:u32)  [unwired: 1 in, 1 out]
        n100 = Multiply(x=0.049, y=w391) -> (x*y=w389:dbl)
        n101 = Greater?(x=w385, y=w389) -> (0:w388:bool)
        n102 = case "Bug: actually, not working" shown="True" w388 {
          tunnel: w394 -> [w405 w408]
          tunnel: [w405 w407] -> w393
          tunnel: w385 -> [_ w406]
          tunnel: w387 -> [w404 _]
          tunnel: w384 -> [w403 _]
          frame False {
            n103 = property class="DigNum (strict)"(reference=w404, "Value"=w403) -> ()  [unwired: 1 in, 2 out]
          }
          frame True {
            n104 = Bundle By Name(cluster=w408, "DisplayIncrement"=w406) -> (w407:T1)
          }
        }
      }
      frame "ChangeRepRate" {
        n105 = Unbundle By Name(w420) -> ("DisplayIncrementRef"=w409:refnum<vi>, "DisplayIncrement"=w412:u32, "CmdParams."=w416:variant)
        n106 = Variant To Data(type=0.0 ("Rep .Rate (Hz)"), Variant=w416) -> (data=w410:dbl)  [unwired: 1 in, 1 out]
        n107 = Bundle By Name(cluster=w420, "Rep .Rate (Hz)"=w410) -> (w419:T1)
        n108 = Multiply(x=0.049, y=w410) -> (x*y=w413:dbl)
        n109 = Greater?(x=w413, y=w412) -> (0:w411:bool)
        n110 = case shown="True" w411 {
          tunnel: w419 -> [w429 w436]
          tunnel: [w429 w435] -> w415
          tunnel: w410 -> [_ w434]
          tunnel: w409 -> [_ w432]
          frame False {
          }
          frame True {
            n111 = Divide(x=w434, y=10.0) -> (x/y=w431:dbl)
            n112 = Round Toward +Infinity(x=w431) -> (ceil(x): smallest int >= x=w430:dbl)
            n113 = property class="DigNum (strict)"(reference=w432, "Value"=w430) -> ()  [unwired: 1 in, 2 out]
            n114 = Bundle By Name(cluster=w436, "DisplayIncrement"=w430) -> (w435:T1)
          }
        }
      }
      frame "SetWriterRef" {
        w444 = T12 0 items=["no dialog", "OK message", "continue or stop message", "OK message + warnings", "continue/stop + warnings"] ("type of dialog (OK msg:1)")
        w447 = 1 items=["no exception", "cancel error on match", "set error on match"] ("[exception action] (none:0)")
        w450 = u32 0 ("t")
        n115 = flat-sequence {
          tunnel: [w472] -> w453
          tunnel: w452 -> [w464]
          tunnel: w451 -> [w471]
          tunnel: [w465] -> w448
          tunnel: [w460] -> w439
          tunnel: [w459] -> w438
          frame #0 {
            n116 = Unbundle By Name(w471) -> ("WriterQueue"=w467:refnum<queue>, "CmdParams."=w468:variant)
            n117 = Bundle("WriterQueue"=w467, "feedback queue"=refnum<queue> refnum) -> (w470:T13)  [unwired: 1 in]
            n118 = Variant To Data(error in=w464, type=w470, Variant=w468) -> (data=w469:T13, error out=w460:errorcluster)
            n119 = Variant To Data(error in=w464, type=w467, Variant=w468) -> (data=w463:refnum<queue>, error out=w459:errorcluster)
            n120 = Unbundle(w469) -> ("WriterQueue"=w462:refnum<queue>, "feedback queue"=w465:refnum<queue>)
            n121 = Select(t=w462, s=w459, f=w463) -> (s? t:f=w461:refnum<queue>)
            n122 = Bundle By Name(cluster=w471, "WriterQueue"=w461) -> (w472:T1)
          }
        }
        n123 = Merge Errors(w439, w438) -> (w437:errorcluster)
        n124 = And(x=w439, y=w438) -> (x .and. y?=w440:bool)
        n125 = Enqueue Element(queue=w448, element="SetWriter_Done", error in (no error)=w439) -> (error out=w443:errorcluster)  [unwired: 1 in, 2 out]
        n126 = call <vilib>:"General Error Handler.vi"("type of dialog (OK msg:1)"=w444, "error in (no error)"=w443, "[exception action] (none:0)"=w447, "[exception code]"=91) -> ("error out"=w441:errorcluster)  [unwired: 7 in, 4 out]
        n127 = Select(t=w437, s=w440, f=w441) -> (s? t:f=w442:errorcluster)
      }
      frame "Quit" {
      }
    }
  }
  "error out" <- w4
